vi "SC Choose Version.vi"(9 "tool lines":string[](array[string]), 10 "deploying?":bool=TRUE) -> (1 "choice":string)   [LabVIEW 2023]
doc: "When the robot runs a version the project doesn't have: shows what each choice keeps and discards and returns choice = robot (replace mine with the robot's), mine (deploy mine in place of the robot's; deploying only), merge, or empty when the user cancels, keeps theirs while fetching, or closes the window. Reads the systemcore-deploy DIVERGED tool lines (TARGET, ROBOT_DEPLOY, LOCAL_ONLY, ROBOT_ONLY, MERGE_CONFLICT)."
uses:
  <vilib>/Utility/error.llb/Trim Whitespace One-Sided.vi
panel:
  in  "Cancel":bool
  in  "Merge":bool
  in  "Use mine":bool
  in  "Use the robot's":bool
  out "Merge choice":i32(listbox)
  out "Merge text":string caption="Merge: keep both"
  out "Mine choice":i32(listbox)
  out "Mine text":string caption="Use mine in place of the robot's"
  out "Robot choice":i32(listbox)
  out "Robot text":string caption="Replace mine with the latest from the robot"
  out "Intro":string
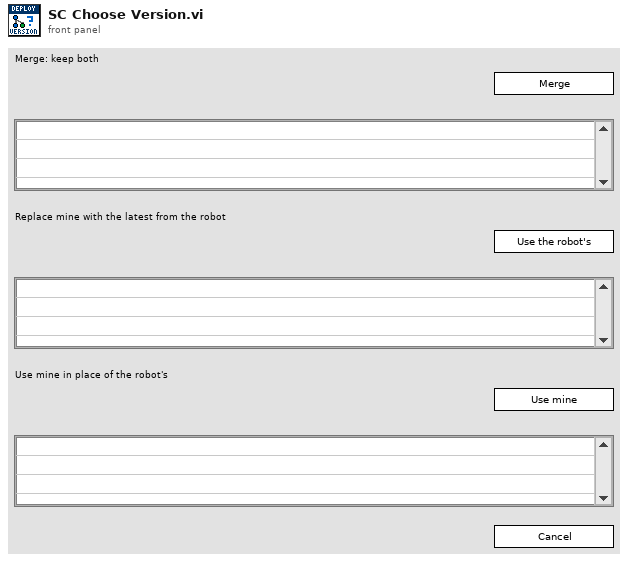
[diagram p1: front panel]
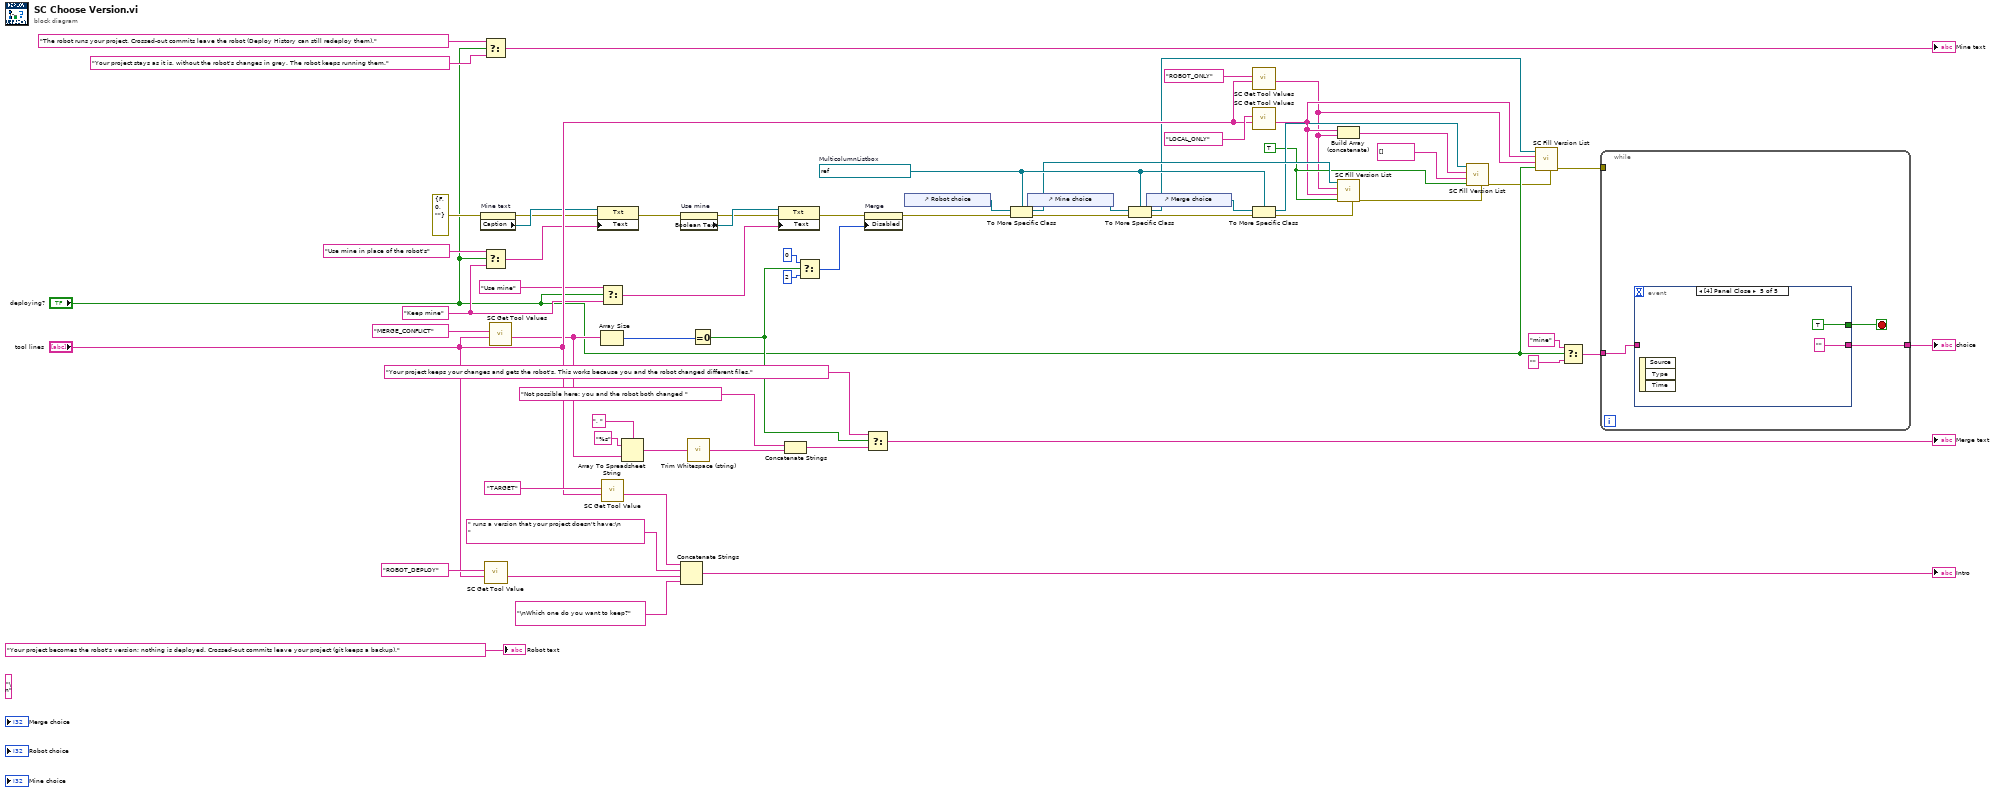
[diagram p0: block diagram]
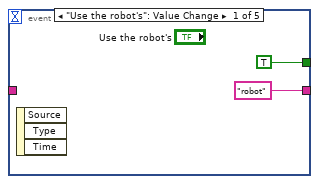
[diagram p2: hidden frame]
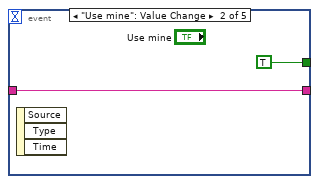
[diagram p3: hidden frame]
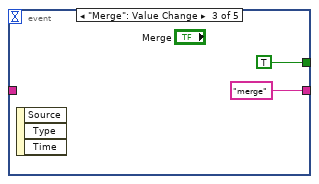
[diagram p4: hidden frame]
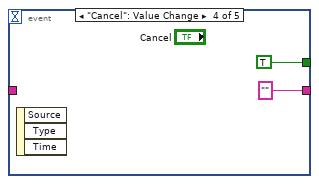
[diagram p5: hidden frame]
diagram:
  w10 = TRUE
  w17 = refnum<vi> refnum  # MulticolumnListbox
  w35 = "Keep mine"
  (unwired) "\n"
  n1 = property on="Mine text" class="Str"(error in=errorcluster {"status"=FALSE, "code"=0, "source"=""}) -> (error out=w30:errorcluster, "Caption"=w31:refnum<vi>)  [unwired: 1 in, 1 out]
  n2 = Select(t="The robot runs your project. Crossed-out commits leave the robot (Deploy History can still redeploy them).", s="deploying?", f="Your project stays as it is, without the robot's changes in grey. The robot keeps running them.") -> (s? t:f=→"Mine text":string)
  n3 = Select(t="Use mine in place of the robot's", s="deploying?", f=w35) -> (s? t:f=w29:string)
  n4 = call "SC Get Tool Value.vi"("tool lines"="tool lines", "key"="ROBOT_DEPLOY") -> ("value"=w61:string)  [unwired: 8 in, 1 out]
  n5 = call "SC Get Tool Values.vi"("tool lines"="tool lines", "key"="MERGE_CONFLICT") -> ("values"=w47:string[])  [unwired: 9 in]
  n6 = property class="Txt"(reference=w31, error in=w30, "Text"=w29) -> (error out=w28:errorcluster)  [unwired: 1 out]
  n7 = Array Size(array=w47) -> (size(s)=w46:i32)
  n8 = Select(t="Use mine", s="deploying?", f=w35) -> (s? t:f=w25:string)
  n9 = call "SC Get Tool Value.vi"("tool lines"="tool lines", "key"="TARGET") -> ("value"=w63:string)  [unwired: 8 in, 1 out]
  n10 = Array To Spreadsheet String(delimiter (Tab)=", ", array=w47, 3:"%s") -> (spreadsheet string=w48:string)
  n11 = Concatenate Strings(w63, " runs a version that your project doesn't have:\n    ", w61, "\nWhich one do you want to keep?") -> (→"Intro":string)
  n12 = property on="Use mine" class="Bool"(error in=w28) -> (error out=w26:errorcluster, "Boolean Text"=w27:refnum<vi>)  [unwired: 1 in, 1 out]
  n13 = call <vilib>:"Trim Whitespace (string).vi"("string"=w48) -> ("trimmed string"=w44:string)  [unwired: 1 in]
  n14 = Equal To 0?(x=w46) -> (x = 0?=w40:bool)
  n15 = property class="Txt"(reference=w27, error in=w26, "Text"=w25) -> (error out=w24:errorcluster)  [unwired: 1 out]
  n16 = Concatenate Strings("Not possible here: you and the robot both changed ", w44) -> (w42:string)
  n17 = Select(t=u8 0, s=w40, f=u8 2) -> (s? t:f=w23:u8)
  n18 = property on="Merge" class="Bool"(error in=w24, "Disabled"=w23) -> (error out=w21:errorcluster)  [unwired: 1 in, 1 out]
  n19 = Select(t="Your project keeps your changes and gets the robot's. This works because you and the robot changed different files.", s=w40, f=w42) -> (s? t:f=→"Merge text":string)
  n20 = control-ref of="Robot choice"() -> (w22:refnum<vi>)
  n21 = To More Specific Class(target class=w17, reference=w22, error in=w21) -> (specific class reference=w15:refnum<vi>, error out=w19:errorcluster)
  n22 = control-ref of="Mine choice"() -> (w20:refnum<vi>)
  n23 = To More Specific Class(target class=w17, reference=w20, error in=w19) -> (specific class reference=w8:refnum<vi>, error out=w16:errorcluster)
  n24 = control-ref of="Merge choice"() -> (w18:refnum<vi>)
  n25 = call "SC Get Tool Values.vi"("tool lines"="tool lines", "key"="ROBOT_ONLY") -> ("values"=w6:string[])  [unwired: 9 in]
  n26 = call "SC Get Tool Values.vi"("tool lines"="tool lines", "key"="LOCAL_ONLY") -> ("values"=w7:string[])  [unwired: 9 in]
  n27 = To More Specific Class(target class=w17, reference=w18, error in=w16) -> (specific class reference=w13:refnum<vi>, error out=w14:errorcluster)
  n28 = Build Array (concatenate)(w7, w6) -> (w12:string[])
  n29 = call "SC Fill Version List.vi"("error in (no error)"=w14, "others discarded?"=w10, "others"=w7, "keeps"=w6, "list"=w15) -> ("error out"=w9:errorcluster)  [unwired: 6 in]
  n30 = call "SC Fill Version List.vi"("error in (no error)"=w9, "others discarded?"=w10, "others"=string[] [], "keeps"=w12, "list"=w13) -> ("error out"=w4:errorcluster)  [unwired: 6 in]
  n31 = call "SC Fill Version List.vi"("error in (no error)"=w4, "others discarded?"="deploying?", "others"=w6, "keeps"=w7, "list"=w8) -> ("error out"=w3:errorcluster)  [unwired: 6 in]
  n32 = Select(t="mine", s="deploying?", f="") -> (s? t:f=w2:string)
  n33 = while {
    tunnel: w3 -> [_]
    tunnel: w2 -> [w68]
    tunnel: [w66] -> w1
    stop <- w67 stop-if-true
    n34 = event shown="[4] Panel Close" {
      selector: _ -> [_ _ _ _ _]
      dyn-events: _ -> [_ _ _ _ _]
      timeout: _ -> [_ _ _ _ _]
      tunnel: w68 -> [_ w71 _ _ _]
      tunnel: [TRUE TRUE TRUE TRUE TRUE] -> w67
      tunnel: ["robot" w71 "merge" "" ""] -> w66
      event "Use the robot's": Value Change {
        n35 = event-data() -> ()  [unwired: 1 in, 3 out]
      }
      event "Use mine": Value Change {
        n36 = event-data() -> ()  [unwired: 1 in, 3 out]
      }
      event "Merge": Value Change {
        n37 = event-data() -> ()  [unwired: 1 in, 3 out]
      }
      event "Cancel": Value Change {
        n38 = event-data() -> ()  [unwired: 1 in, 3 out]
      }
      event Panel Close {
        n39 = event-data() -> ()  [unwired: 1 in, 3 out]
      }
    }
  }
  "choice" <- w1
  "Robot text" <- "Your project becomes the robot's version; nothing is deployed. Crossed-out commits leave your project (git keeps a backup)."
